vi "Call Function.vi"(6 "Input String":string, 8 "error in":errorcluster, 9 "Function":string, 10 "Python Script":path, 11 "IPython Caller in":refnum<class "IPython Caller.lvclass">) -> (0 "error out":errorcluster, 2 "Return String":string, 3 "IPython Caller out":refnum<class "IPython Caller.lvclass">)   [LabVIEW 2026, in "IPython Caller.lvclass"]
doc: "This VI calls the specified function from a python script. This VI can only call functions with a string input and output parameter. The function uses the tool global virtual environment."
uses:
  IPython Caller.lvclass
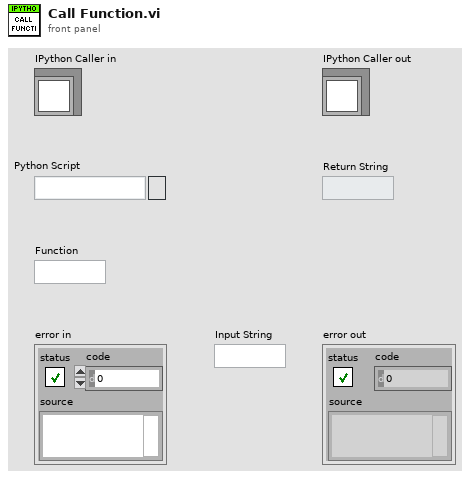
[diagram p1: front panel]
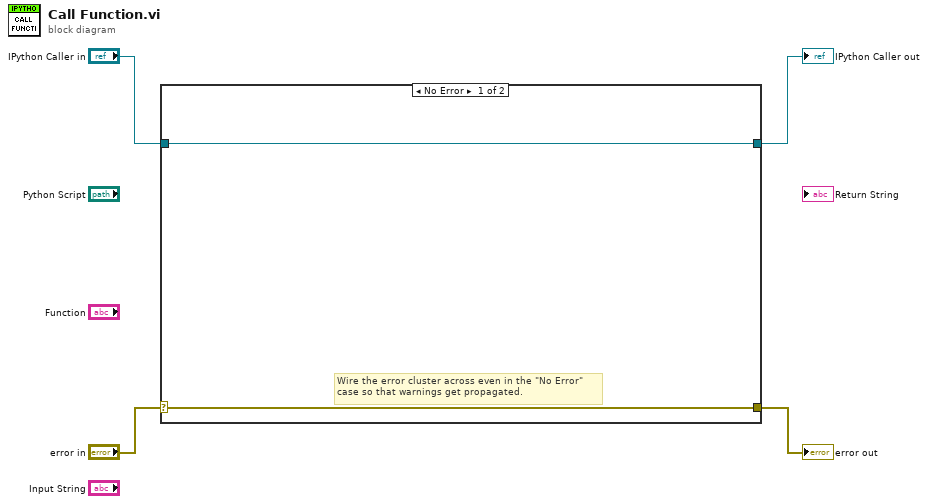
[diagram p0: block diagram]
diagram:
  n1 = case shown="No Error" "error in" {
    selector: "error in" -> [w6 w8]
    tunnel: [w6 w8] -> w3
    tunnel: [w5 w7] -> w1
    tunnel: "IPython Caller in" -> [w5 w7]
    frame No Error {
      # "Wire the error cluster across even in the \"No Error\"\ncase so that warnings get propagated."
    }
    frame Error {
    }
  }
  "error out" <- w3
  "IPython Caller out" <- w1
